vi "LHF.DB.Mongo.Collection.Find.vi"(6 "Extract _id":bool=TRUE, 7 "document type":variant, 8 "error in (no error)":errorcluster, 9 "query":variant, 10 "Collection":string, 11 "LHF.DB.Mongo in":refnum<class "LHF.DB.Mongo.lvclass">) -> (0 "error out":errorcluster, 1 "ObjectIDs":string[](array[string]), 2 "Documents":variant[](array[variant]), 3 "LHF.DB.Mongo out":refnum<class "LHF.DB.Mongo.lvclass">)   [LabVIEW 2013, in "LHF.DB.Mongo.lvclass"]
doc: "Query: use clusters named with query operation (if none, equal is used) or a Query.NET object. If a single field is being queried, you may it by setting the variable name as the field name in database. \nYou may use <, <=, >, >=, ==, !=, and others in variables name to choose operation, and you may aggregate them by putting in a cluster with $and or $or."
uses:
  LHF.DB.Mongo.lvclass
  C:/Users/Ricardo/Desktop/Projetos/LabVIEW-MongoDB/src/Driver/MongoDB.Driver.dll
  Driver/MongoDB.Driver.dll
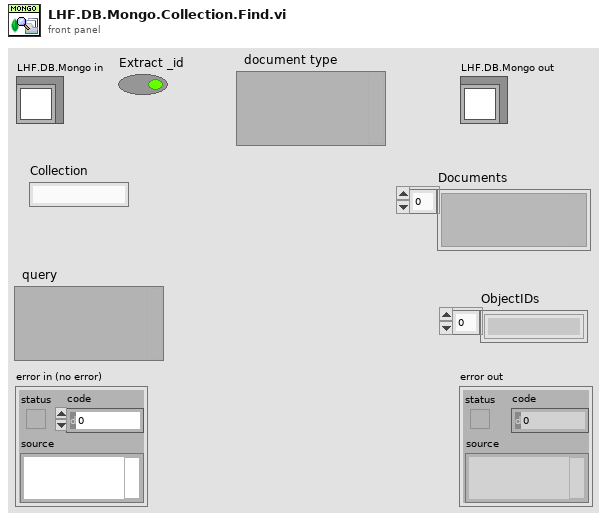
[diagram p1: front panel]
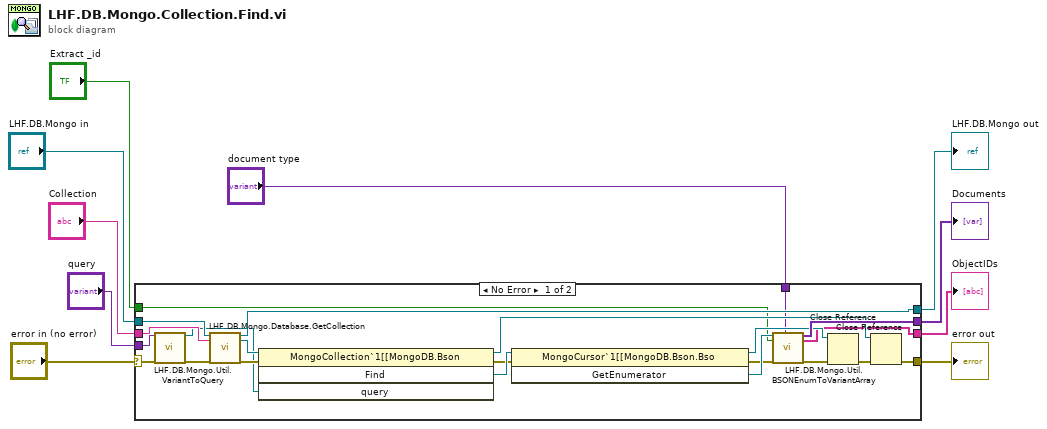
[diagram p0: block diagram]
diagram:
  n1 = case shown="No Error" "error in (no error)" {
    selector: "error in (no error)" -> [w13 w34]
    tunnel: [w21 w34] -> w9
    tunnel: [w31 w33] -> w7
    tunnel: "LHF.DB.Mongo in" -> [w30 w33]
    tunnel: "Collection" -> [w32 _]
    tunnel: [w27 _] -> w5
    tunnel: "query" -> [w18 _]
    tunnel: [w16 _] -> w3
    tunnel: "Extract _id" -> [w15 _]
    tunnel: "document type" -> [w11 _]
    frame No Error {
      n2 = call "LHF.DB.Mongo.Util.VariantToQuery.vi"("Equal"=w18, "error in (no error)"=w13) -> (".NET Refnum out"=w14:refnum<k24>, "error out"=w12:errorcluster)  [unwired: 16 in]
      n3 = call "LHF.DB.Mongo.Database.GetCollection.vi"("LHF.DB.Mongo in"=w30, "collectionName"=w32, "error in (no error)"=w12) -> ("LHF.DB.Mongo in"=w31:refnum<class "LHF.DB.Mongo.lvclass">, "MongoCollection"=w19:refnum<k24>, "error out"=w17:errorcluster)  [unwired: 14 in]
      n4 = invoke class="MongoCollection`1[[MongoDB.Bson" method="Find"(reference=w19, error in=w17, "query"=w14) -> (reference out=w23:refnum<k24>, error out=w25:errorcluster, "Find"=w29:refnum<k24>)  [unwired: 1 in, 1 out]
      n5 = invoke class="MongoCursor`1[[MongoDB.Bson.Bso" method="GetEnumerator"(reference=w29, error in=w25) -> (reference out=w24:refnum<k24>, error out=w26:errorcluster, "GetEnumerator"=w28:refnum<k24>)  [unwired: 1 in]
      n6 = call "LHF.DB.Mongo.Util.BSONEnumToVariantArray.vi"("BsonENUM"=w28, "Extract _id"=w15, "error in (no error)"=w26, "type"=w11) -> ("Documents"=w27:variant[], "ObjectIDs"=w16:string[], "error out"=w20:errorcluster)  [unwired: 13 in]
      n7 = Close Reference(reference=w24, error in (no error)=w20) -> (error out=w22:errorcluster)
      n8 = Close Reference(reference=w23, error in (no error)=w22) -> (error out=w21:errorcluster)
    }
    frame Error {
    }
  }
  "error out" <- w9
  "LHF.DB.Mongo out" <- w7
  "Documents" <- w5
  "ObjectIDs" <- w3
